vi "lvmcp_delete.vi"() -> ()   [LabVIEW 2026]
panel:
  in  "References":refnum<vi>[](array[refnum])
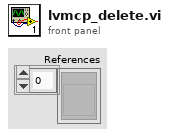
[diagram p1: front panel]
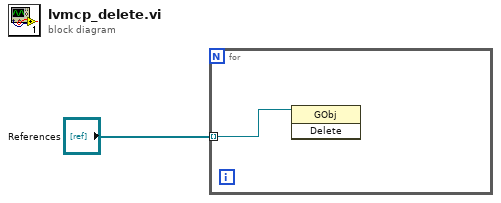
[diagram p0: block diagram]
diagram:
  n1 = for {
    tunnel: "References" -> [w2] mode=indexing
    n2 = invoke class="GObj" method="Delete"(reference=w2) -> ()  [unwired: 2 in, 3 out]
  }
